vi "synchronize_mnu_file_with_directory.vi"(8 "error in (no error)":errorcluster, 9 "Synchronized Directory":path, 10 "MNU File":path, 11 "Unpacked Package Directory":path) -> (0 "error out":errorcluster)   [LabVIEW 2020, in "vi_package_building_extensions.lvlib"]
uses:
  vi_package_building_extensions.lvlib
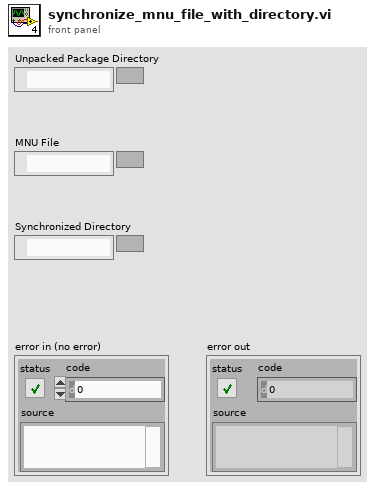
[diagram p1: front panel]
types:
  T1 = typedef "Palette Menu.lvlib/Palette Data.ctl" = cluster{"display name":string, "view format":T2, "palette width":i16, "items":T3, "256 color icon":picture, "B&W color icon":picture, "help information":T5, "palette description":string, "synchronize information":T6}
  T2 = typedef "Palette Menu.lvlib/View Format.ctl" = u16
  T3 = typedef "Palette Menu.lvlib/Items.ctl" = T4[]
  T4 = typedef "Palette Menu.lvlib/Item.ctl" = cluster{"item path":path, "library path":path, "use default lvlib palette":bool, "short name":string, "place VI contents":bool, "hide synchronized item":bool, "reserve spot for synch item":bool, "configure when placing VI contents":bool}
  T5 = typedef "Palette Menu.lvlib/Help Info.ctl" = cluster{"help tag":string, "help file path ":path}
  T6 = typedef "Palette Menu.lvlib/Synchronize Info.ctl" = cluster{"synchronize with directory":bool, "synchronize directory path":path}
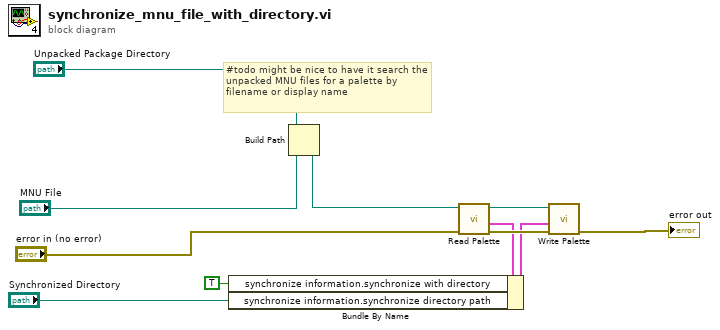
[diagram p0: block diagram]
diagram:
  # "#todo might be nice to have it search the unpacked MNU files for a palette by filename or display name"
  n1 = Build Path(base path="Unpacked Package Directory", name or relative path="MNU File") -> (appended path=w10:path)
  n2 = call <vilib>:"Read Palette.vi"("error in (no error)"="error in (no error)", "palette path"=w10) -> ("error out"=w8:errorcluster, "palette data"=w5:T1, "duplicate palette path"=w4:path)  [unwired: 7 in]
  n3 = Bundle By Name(cluster=w5, "synchronize information.synchronize with directory"=TRUE, "synchronize information.synchronize directory path"="Synchronized Directory") -> (w6:T1)
  n4 = call <vilib>:"Write Palette.vi"("error in (no error)"=w8, "palette data"=w6, "palette path"=w4) -> ("error out"=→"error out":errorcluster)  [unwired: 8 in]
